vi "PicoScope3000aExampleEts.vi"() -> ()   [LabVIEW 2010]
uses:
  shared/PicoBuffers.ctl
  shared/Buffer and Transfer Settings.ctl
  shared/Acquisition Settings.ctl
  PicoScope3000aLib/PicoScope3000aAnalogChannelSettings.ctl
panel:
  out "Properties Panel":T1 {"Max Total Capture Time Available (sec)" format="%.3p"; "Sample Frequency" format="%.3p"; "Sample Rate" format="%.3p"; "Max Samples Available" format="%.3p"; "Total Capture Time (sec)" format="%.3p"}
  out "EtsTimeValues":i64[](array[numeric])
  in  "etsInterleave":i16=40
  in  "etsCycles":i16=200
  out "Max etsInterleave":i16
  out "Max etsCycles":i16
  in  "Trigger Settings":T2={"Trigger Enabled"=TRUE, "Trigger Source"=enum."Channel A", "Trigger Threshold (volts)"=0.0, "Trigger Direction"=2, "Trigger Delay (samples)"=0, "Auto Trigger Time (ms)"=1000} {"Trigger Direction" items=["Above", "Below", "Rising", "Falling", "Rising or Falling"]}
  in  "ETS Mode":u32(ring)=1 items=["PS3000A_ETS_OFF", "PS3000A_ETS_FAST", "PS3000A_ETS_SLOW"]
  in  "Channel A Settings":T3={"Enabled"=TRUE, "Coupling"=1, "Range"=6, "Analogue Offset"=0.0, "Bandwidth Limit"=0} {"Bandwidth Limit" items=["Full", "20MHz"]; "Range" items=["10 mV", "20 mV", "50 mV", "100 mV", "200 mV", "500 mV", "1 V", "2 V", "5 V", "10 V", "20 V", "50 V ", "100 V"]; "Coupling" items=["AC", "DC"]}
  out "overflow":i16 format="%010b"
  in  "Apply Settings":bool
  out "USB 3.0 device on non-USB 3.0 Port":bool=TRUE
  out "USB Powered":bool=TRUE
  out "Device Info":T4={"Driver Version"="0", "USB Version"="0", "Hardware"="0", "Variant"="0", "Batch and Serial"="0", "Cal Date"="0", "Kernel Version"="0", "Digital HW Version"="0", "Analogue HW Version"="0", "MSO"=FALSE, "Number of channels"=0}
  out "error out":errorcluster
  in  "Data file":path=path "PicoScope3000aExampleETS ChA Data"
  in  "Buffer and Transfer Settings":T5={"startIndex"=0, "Samples"=1000, "Down Sample Ratio"=1, "Down-Sample Mode"=0} {"Down-Sample Mode" items=["RAW none"=2147483648, "None"=0, "Aggregate"=1, "Decimate"=2, "Average"=4]; "Down Sample Ratio" step=1; "Samples" format="%_6p"}
  in  "Acquisition Settings":T6={"preTriggerSamples"=0, "postTriggerSamples"=1000, "timebase"=0} {"postTriggerSamples" format="%_6p"; "preTriggerSamples" format="%_6p"}
  in  "stop":bool
  out "Channel A":cluster{i32, sgl, "Data":dbl[]}(graph)
  in  "Serial Number":string
  in  "Use Serial Number":bool
  in  "error in (no error)":errorcluster
  # "Bit 0 = ChA"
  # "ETS mode on channel A only"
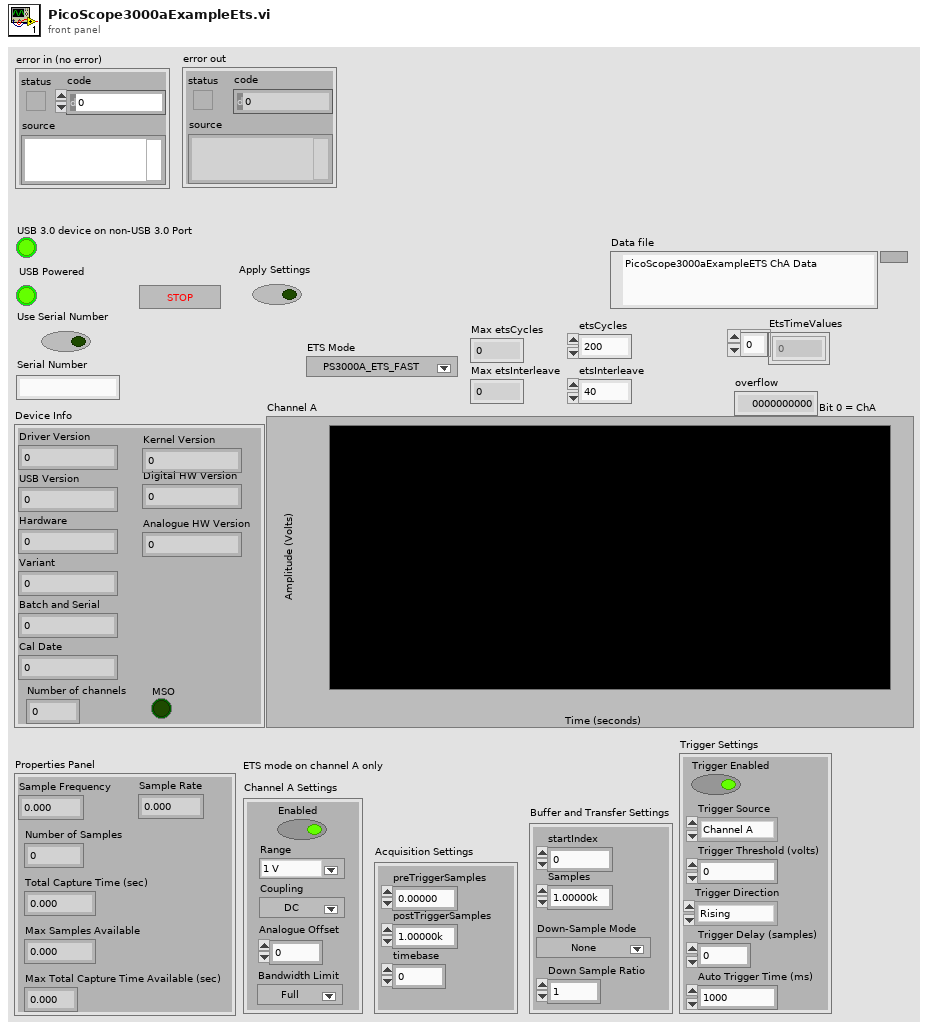
[diagram p1: front panel]
types:
  T1 = cluster{"Sample Frequency":sgl, "Sample Rate":sgl, "Max Samples Available":i32, "Number of Samples":u32, "Total Capture Time (sec) ":sgl, "Max Total Capture Time Available (sec)":sgl}
  T2 = cluster{"Trigger Enabled":bool, "Trigger Source":enum32{"Channel A", "Channel B", "Channel C", "Channel D", "Ext."}, "Trigger Threshold (volts)":dbl, "Trigger Direction":u32, "Trigger Delay (samples)":u32, "Auto Trigger Time (ms)":i16}
  T3 = typedef "PicoScope3000aAnalogChannelSettings.ctl" = cluster{"Enabled":bool, "Coupling":u32, "Range":u32, "Analogue Offset":sgl, "Bandwidth Limit":u32}
  T4 = cluster{"Driver Version":string, "USB Version":string, "Hardware":string, "Variant":string, "Batch and Serial":string, "Cal Date":string, "Kernel Version":string, "Digital HW Version":string, "Analogue HW Version":string, "MSO":bool, "Number of channels":i16}
  T5 = typedef "Buffer and Transfer Settings.ctl" = cluster{"startIndex":u64, "Samples":u64, "Down Sample Ratio":u64, "Down-Sample Mode":u32}
  T6 = typedef "Acquisition Settings.ctl" = cluster{"preTriggerSamples":u64, "postTriggerSamples":u64, "timebase":u32}
  T7 = enum16{"open", "open or create", "create or replace", "create", "open (read-only)"}
  T8 = typedef "PicoBuffers.ctl" = cluster{"Max Buffer Pointers":u64[][][], "Min Buffer Pointers":u64[][][], "StreamingDataInfo":cluster{"Channel":u32, "Down-Sample Mode":u32, "PICO_DATA_TYPE":enum32{"PICO_INT8_T", "PICO_INT16_T", "PICO_INT32_T", "PICO_UINT32_T", "PICO_INT64_T", ""}, "Samples":i32, "bufferIndex":u64, "startIndex":i32, "overflow":i16}[][]}
  T9 = cluster{"Channel A Buffer":i16[], "Channel B Buffer":i16[], "Channel C Buffer":i16[], "Channel D Buffer":i16[], "Channel E Buffer":i16[], "Channel F Buffer":i16[], "Channel G Buffer":i16[], "Channel H Buffer":i16[], "Port 0 Buffer":i16[], "Port 1 Buffer":i16[]}[]
  T10 = cluster{"Channel A Buffer":i16[], "Channel B Buffer":i16[], "Channel C Buffer":i16[], "Channel D Buffer":i16[], "Channel E Buffer":i16[], "Channel F Buffer":i16[], "Channel G Buffer":i16[], "Channel H Buffer":i16[], "Port 0 Buffer":i16[], "Port 1 Buffer":i16[]}
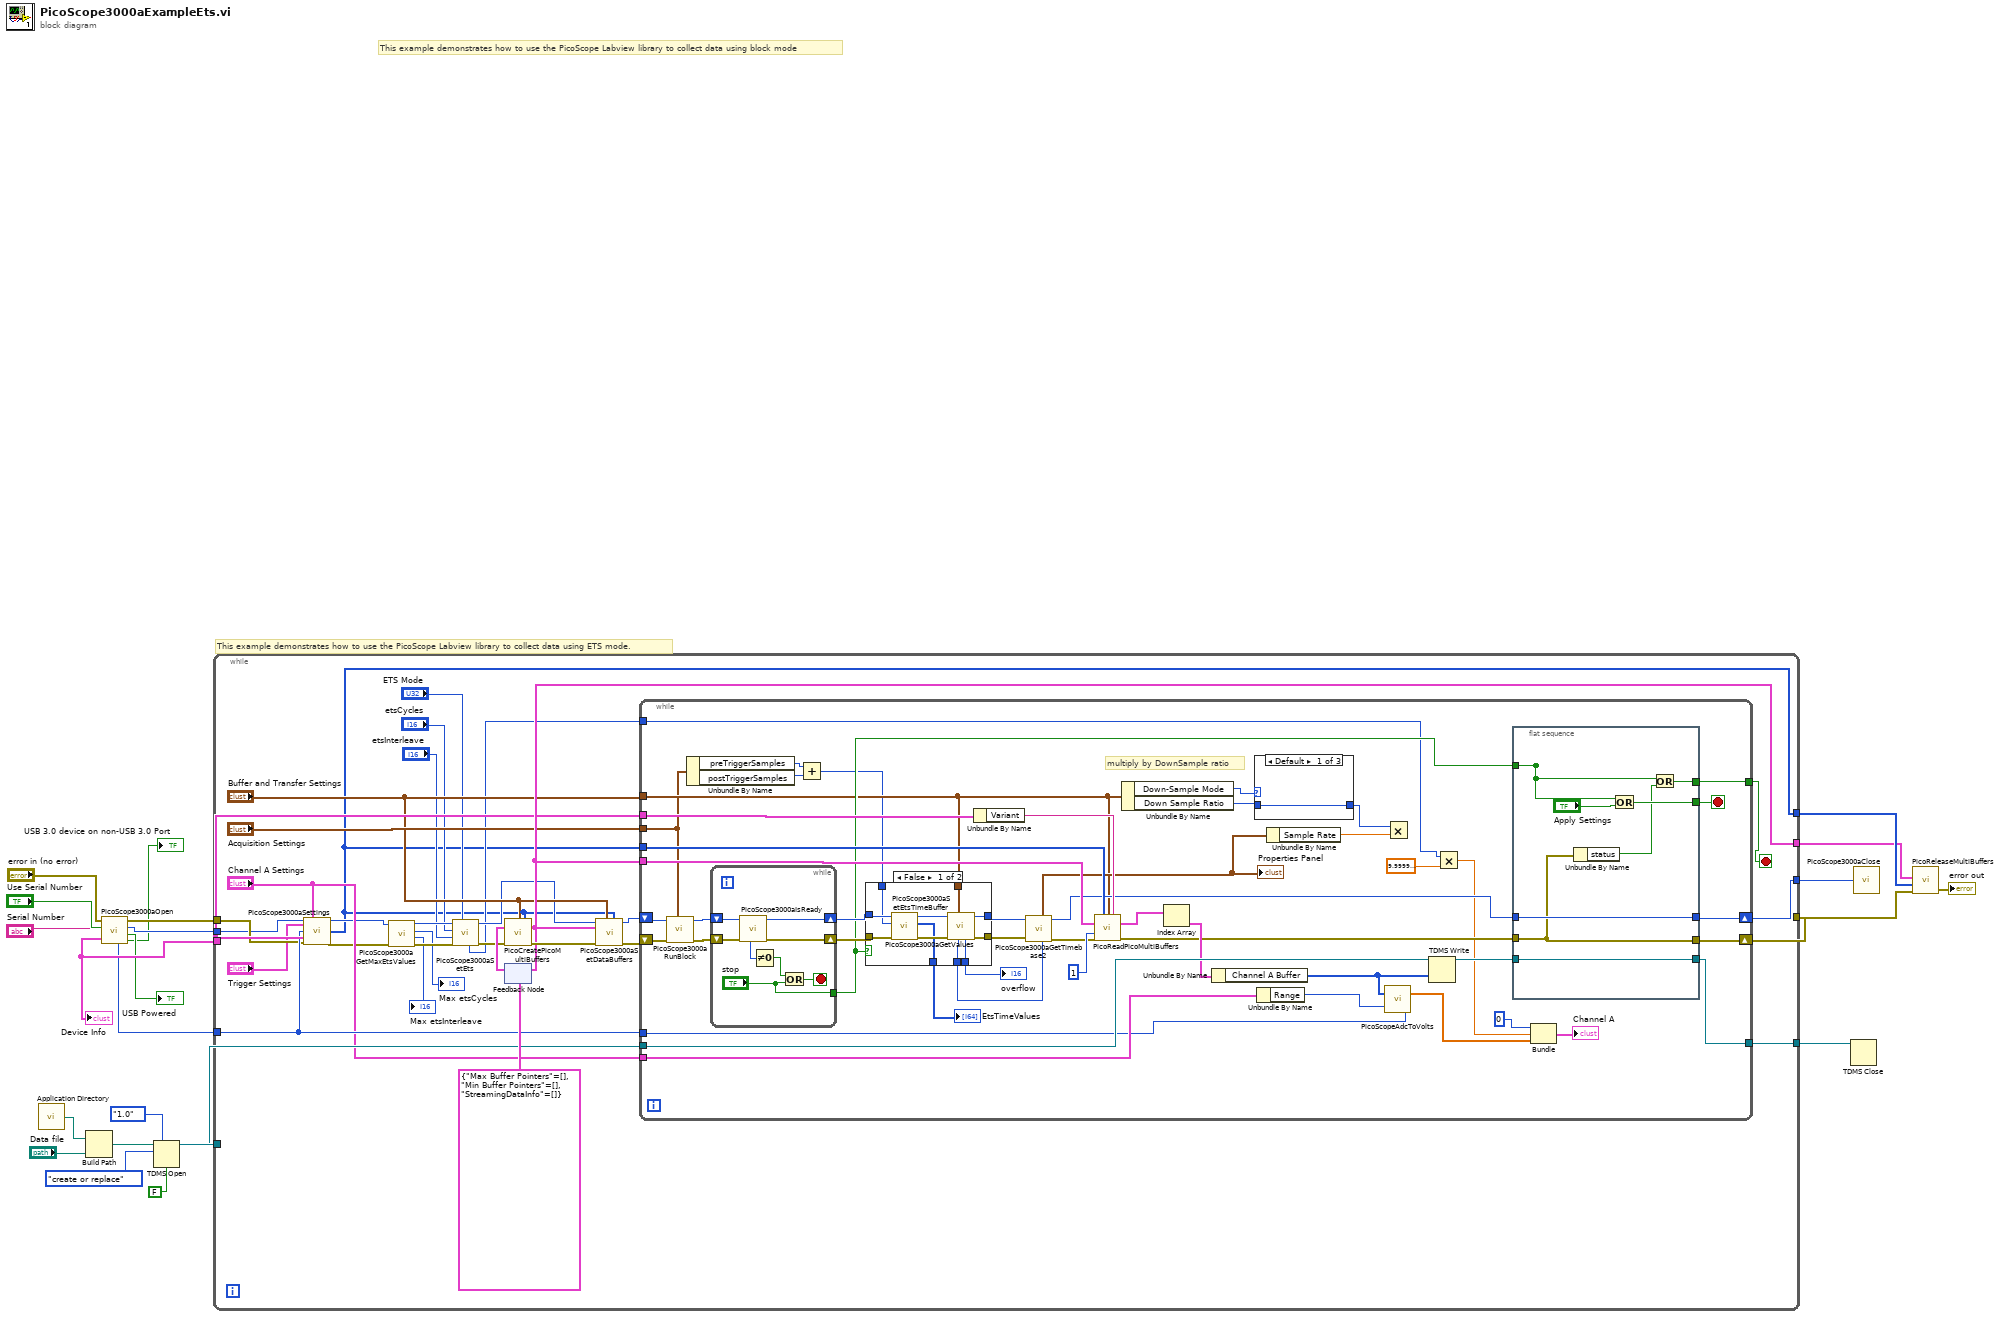
[diagram p0: block diagram]
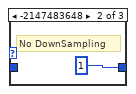
[diagram p3: hidden frame]
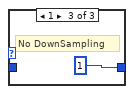
[diagram p4: hidden frame]
diagram:
  # "This example demonstrates how to use the PicoScope Labview library to collect data using ETS mode."
  # "This example demonstrates how to use the PicoScope Labview library to collect data using block mode"
  n1 = call <vilib>:"Application Directory.vi"() -> ("Application Directory"=w14:path)
  n2 = Build Path(base path=w14, name or relative path="Data file") -> (appended path=w15:path)
  n3 = call "PicoScope3000aOpen.vi"("Batch/Serial"="Serial Number", "Use Serial number"="Use Serial Number", "error in (no error)"="error in (no error)") -> ("USB 3.0 device on non-USB 3.0 Port"=→"USB 3.0 device on non-USB 3.0 Port":bool, "USB Powered"=→"USB Powered":bool, "handle"=w22:i16, "error out"=w5:errorcluster, "Max ADC value"=w2:i16, "Device Info"=w7:T4)  [unwired: 3 in]
  "Device Info" <- w7
  n4 = TDMS Open(6:FALSE ("disable buffering? (T)"), 7:enum16{"1.0", "2.0"}."1.0" ("file format version (2.0)"), 10:T7."create or replace" ("operation (0:open)"), 11:w15) -> (3:w12:refnum<k34>)  [unwired: 2 in, 1 out]
  n5 = while {
    tunnel: w22 -> [w26]
    tunnel: w2 -> [w40]
    tunnel: [w24] -> w21
    tunnel: [w51] -> w20
    tunnel: [w46] -> w13
    tunnel: w12 -> [w50]
    tunnel: w7 -> [w48]
    tunnel: w5 -> [w27]
    tunnel: [w47] -> w4
    tunnel: [w44] -> w3
    stop <- w45 stop-if-true
    n6 = call "PicoScope3000aSettings.vi"("handle in"=w26, "Channel A Settings"="Channel A Settings", "Trigger Settings"="Trigger Settings", "Max_adc"=w40, "Device Info"=w48, "error in"=w27) -> ("handle out"=w25:i16, "Enabled Array"=w24:i16[], "error out"=w28:errorcluster)  [unwired: 7 in]
    n7 = call "PicoScope3000aGetMaxEtsValues.vi"("error in (no error)"=w28, "handle in"=w25) -> ("error out"=w38:errorcluster, "Max etsInterleave"=→"Max etsInterleave":i16, "Max etsCycles"=→"Max etsCycles":i16, "handle out"=w35:i16)  [unwired: 6 in]
    n8 = call "PicoScope3000aSetEts.vi"("ETS Mode"="ETS Mode", "error in (no error)"=w38, "etsInterleave"="etsInterleave", "etsCycles"="etsCycles", "handle in"=w35) -> ("error out"=w37:errorcluster, "handle out"=w36:i16, "sampleTimePicoseconds"=w34:i32)  [unwired: 4 in]
    n9 = feedback #1(T8 {"Max Buffer Pointers"=[], "Min Buffer Pointers"=[], "StreamingDataInfo"=[]} ("Data Pointers")) -> (w53:T8)
    n10 = call "PicoCreatePicoMultiBuffers.vi"("Buffer and Transfer Settings"="Buffer and Transfer Settings", "enabled array"=w24, "Data Pointers In"=w53, "error in (no error)"=w37) -> ("Data Pointers"=w51:T8, "error out"=w52:errorcluster)  [unwired: 10 in]
    n11 = feedback-in #1(w51) -> ()
    n12 = call "PicoScope3000aSetDataBuffers.vi"("enabled array"=w24, "Buffer and Transfer Settings"="Buffer and Transfer Settings", "error in (no error)"=w52, "Data Pointers In"=w51, "handle in"=w36) -> ("error out"=w43:errorcluster, "handle out"=w42:i16)  [unwired: 5 in]
    n13 = while {
      tunnel: w51 -> [w103]
      tunnel: "Buffer and Transfer Settings" -> [w65]
      tunnel: w24 -> [w95]
      tunnel: "Channel A Settings" -> [w94]
      tunnel: "Acquisition Settings" -> [w58]
      tunnel: w40 -> [w93]
      tunnel: w48 -> [w90]
      tunnel: [w80] -> w45
      shift-right: [w84] -> w47
      shift-left: w43 -> [w74]
      shift-right: [w78] -> w44
      shift-left: w42 -> [w75]
      tunnel: w50 -> [w102]
      tunnel: [w82] -> w46
      tunnel: w34 -> [w62]
      stop <- w79 stop-if-true
      # "multiply by DownSample ratio"
      n14 = call "PicoScope3000aRunBlock.vi"("Acquisition Settings"=w58, "error in (no error)"=w74, "handle in"=w75) -> ("error out"=w97:errorcluster, "handle out"=w96:i16)  [unwired: 5 in, 2 out]
      n15 = Unbundle By Name(w58) -> ("preTriggerSamples"=w57:u64, "postTriggerSamples"=w56:u64)
      n16 = while {
        shift-right: [w131] -> w76
        shift-left: w97 -> [w132]
        shift-right: [w130] -> w77
        shift-left: w96 -> [w129]
        tunnel: ["stop"] -> w73
        stop <- w126 stop-if-true
        n17 = call "PicoScope3000aIsReady.vi"("error in (no error)"=w132, "handle in"=w129) -> ("error out"=w131:errorcluster, "handle out"=w130:i16, "ready"=w128:i16)  [unwired: 7 in]
        n18 = Not Equal To 0?(x=w128) -> (x != 0?=w127:bool)
        n19 = Or(x=w127, y="stop") -> (x .or. y?=w126:bool)
      }
      n20 = Add(x=w57, y=w56) -> (x+y=w55:u64)
      n21 = case shown="False" w73 {
        tunnel: w76 -> [w109 w115]
        tunnel: w77 -> [w106 w116]
        tunnel: [w114 w116] -> w68
        tunnel: [w113 w115] -> w69
        tunnel: w65 -> [w112 _]
        tunnel: [w111 _] -> w72
        tunnel: [w110 _] -> w71
        tunnel: [w105 _] -> w61
        tunnel: w55 -> [w104 _]
        frame False {
          n22 = call "PicoScope3000aSetEtsTimeBuffer.vi"("error in (no error)"=w109, "bufferLth"=w104, "handle in"=w106) -> ("error out"=w108:errorcluster, "EtsTimeValues"=w105:i64[], "handle out"=w107:i16)  [unwired: 6 in]
          n23 = call "PicoScope3000aGetValues.vi"("Buffer and Transfer Settings"=w112, "error in (no error)"=w108, "handle in"=w107) -> ("error out"=w113:errorcluster, "handle out"=w114:i16, "overflow"=w111:i16, "noOfSamples"=w110:u64)  [unwired: 5 in]
        }
        frame True {
        }
      }
      "overflow" <- w72
      "EtsTimeValues" <- w61
      n24 = Unbundle By Name(w90) -> ("Variant"=w91:string)
      n25 = call "PicoScope3000aGetTimebase2.vi"("Number of Samples"=w71, "error in (no error)"=w69, "handle in"=w68) -> ("error out"=w67:errorcluster, "handle out"=w66:i16, "Properties Panel"=w70:T1)  [unwired: 6 in]
      "Properties Panel" <- w70
      n26 = call "PicoReadPicoMultiBuffers.vi"("enabled array"=w95, "Buffer and Transfer Settings"=w65, "Variant"=w91, "Data Pointers"=w103, "No of Buffers"=1, "error in (no error)"=w67) -> ("MultiBuffers (Max or non-aggregated)"=w101:T9, "error out"=w81:errorcluster)  [unwired: 7 in, 1 out]
      n27 = Unbundle By Name(w65) -> ("Down-Sample Mode"=w99:u32, "Down Sample Ratio"=w100:u64)
      n28 = Index Array(array=w101) -> (element=w85:T10)  [unwired: 1 in]
      n29 = Unbundle By Name(w85) -> ("Channel A Buffer"=w86:i16[])
      n30 = case shown="Default" w99 {
        tunnel: [w133 u64 1 ("Down Sample Ratio") u64 1 ("Down Sample Ratio")] -> w98
        tunnel: w100 -> [w133 _ _]
        frame Default {
        }
        frame -2147483648 {
          # "No DownSampling"
        }
        frame 1 {
          # "No DownSampling"
        }
      }
      n31 = Unbundle By Name(w94) -> ("Range"=w87:u32)
      n32 = Unbundle By Name(w70) -> ("Sample Rate"=w92:sgl)
      n33 = call "PicoScopeAdcToVolts.vi"("Max_adc"=w93, "Range Index"=w87, "Data"=w86) -> ("Data"=w60:dbl[])
      n34 = Multiply(x=w98, y=w92) -> ()  [unwired: 1 out]
      n35 = TDMS Write(0:w102, 9:w86) -> (4:w83:refnum<k34>)  [unwired: 4 in, 3 out]
      n36 = Multiply(x=w62, y=sgl 1e-12) -> (x*y=w63:sgl)
      n37 = flat-sequence {
        tunnel: [w124] -> w79
        tunnel: [w117] -> _
        tunnel: [w121] -> w80
        tunnel: w66 -> [w120]
        tunnel: [w120] -> w78
        tunnel: w81 -> [w119]
        tunnel: [w119] -> w84
        tunnel: [w118] -> w82
        tunnel: w83 -> [w118]
        tunnel: w73 -> [w117]
        frame #0 {
          n38 = Unbundle By Name(w119) -> ("status"=w122:bool)
          n39 = Or(x=w117, y="Apply Settings") -> (x .or. y?=w124:bool)
          n40 = Or(x=w117, y=w122) -> (x .or. y?=w121:bool)
        }
      }
      n41 = Bundle(0, w63, "Data"=w60) -> (→"Channel A":cluster{i32, sgl, "Data":dbl[]})  [unwired: 1 in]
    }
  }
  n42 = TDMS Close(11:w13) -> ()  [unwired: 1 in, 2 out]
  n43 = call "PicoScope3000aClose.vi"("handle"=w3) -> ()
  n44 = call "PicoReleaseMultiBuffers.vi"("error in (no error)"=w4, "Enabled array"=w21, "Data Pointers"=w20) -> ("error out"=→"error out":errorcluster)  [unwired: 8 in]
